vi "CheckDayPassing.vi"(8 "error in":errorcluster, 10 "Data2save.time":dbl[](array[numeric]), 11 "TableName":string) -> (0 "error out":errorcluster, 1 "split-index":i32, 2 "Split array":bool, 3 "FolderPace":T1, 4 "TimeValid":bool, 5 "PeriodName2":string, 7 "PeriodName1":string)   [LabVIEW 2020, in "Sgraph_lib_V1.lvlib" / "DBAL-BIN.lvclass"]
doc: "This VI will check if the time of the dataset is passing one period.\nIf that is the case, then the dataset has to be split in two subsections and processed separately.\n\nAlthough the name of this routine is called 'DayPassing' this was later changed to 'one week' or 'one year' for other file types. Therefore this VI actually checks if the period is passed for which a new file is needed."
uses:
  DBAL-BIN.lvclass
  BinFolderPace.ctl
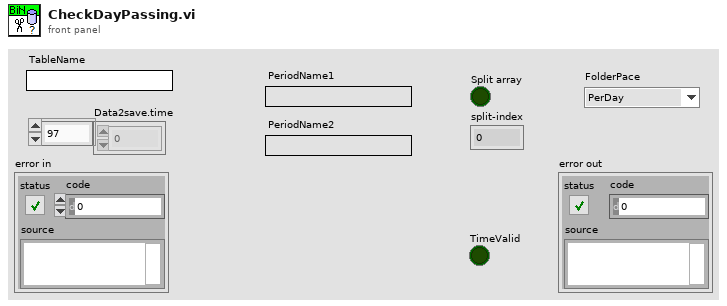
[diagram p1: front panel]
types:
  T1 = typedef "Sgraph_lib_V1.lvlib/DBAL-BIN.lvclass/BinFolderPace.ctl" = enum16{"PerDay", "PerWeek", "PerYear"}
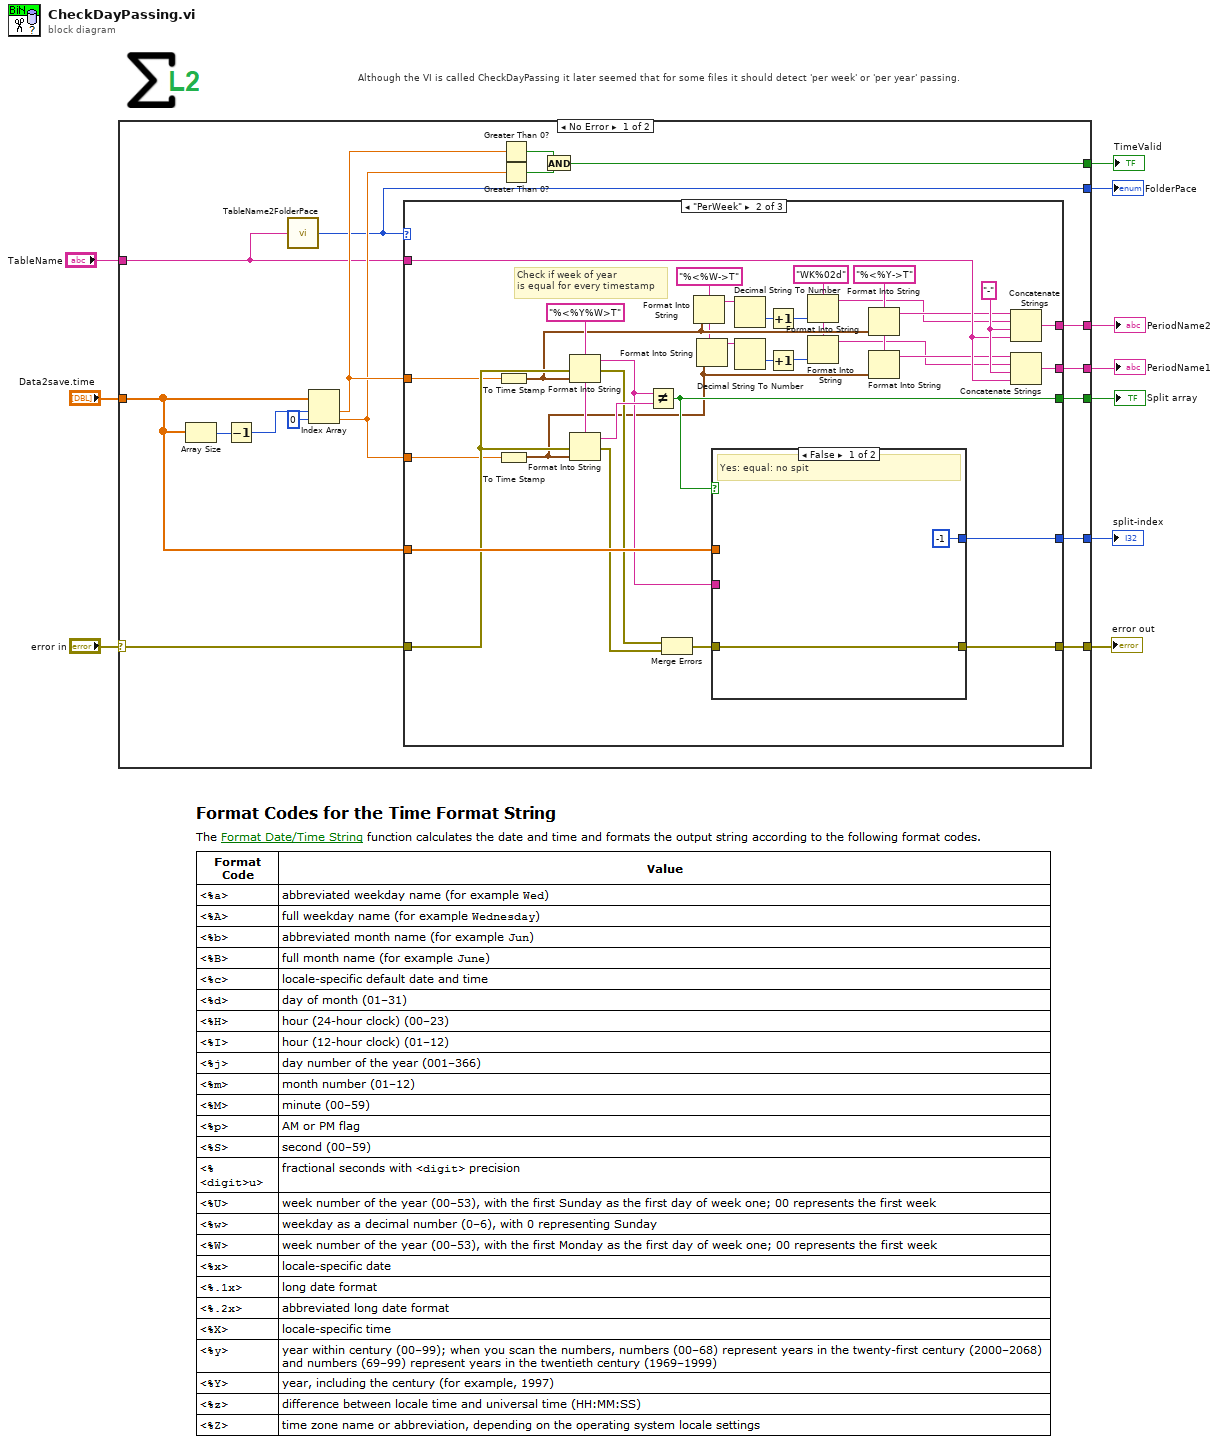
[diagram p0: block diagram]
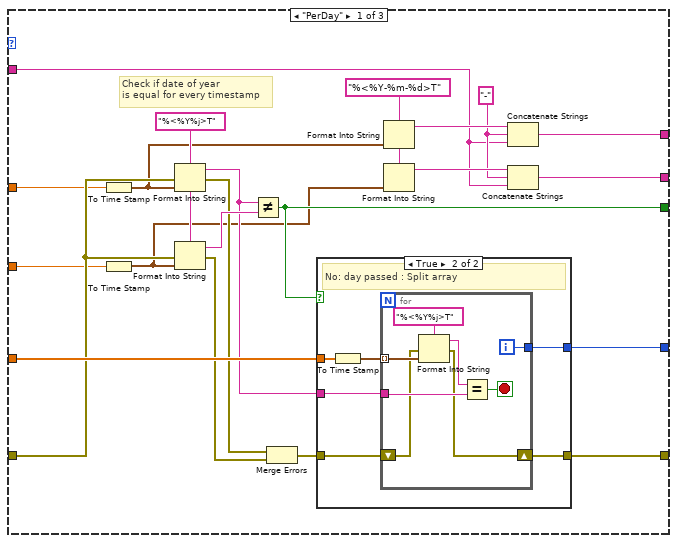
[diagram p2: hidden frame]
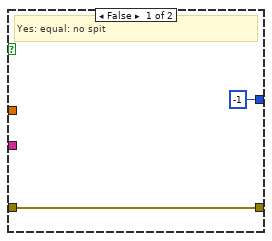
[diagram p3: hidden frame]
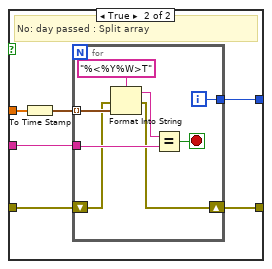
[diagram p4: hidden frame]
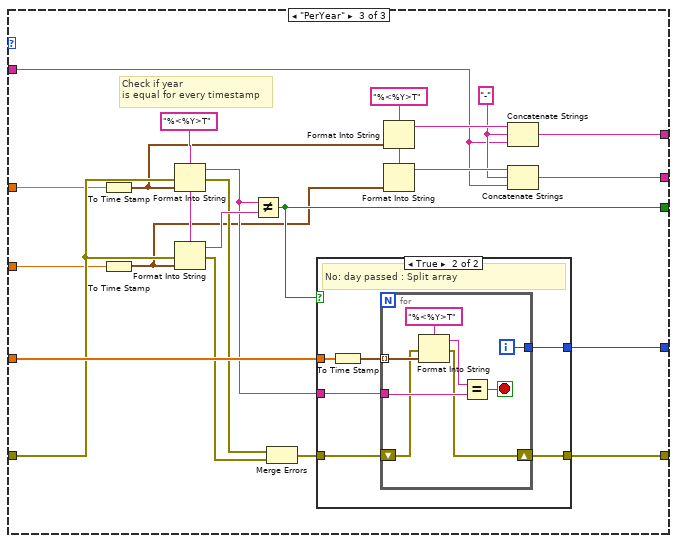
[diagram p5: hidden frame]
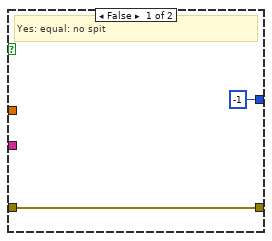
[diagram p6: hidden frame]
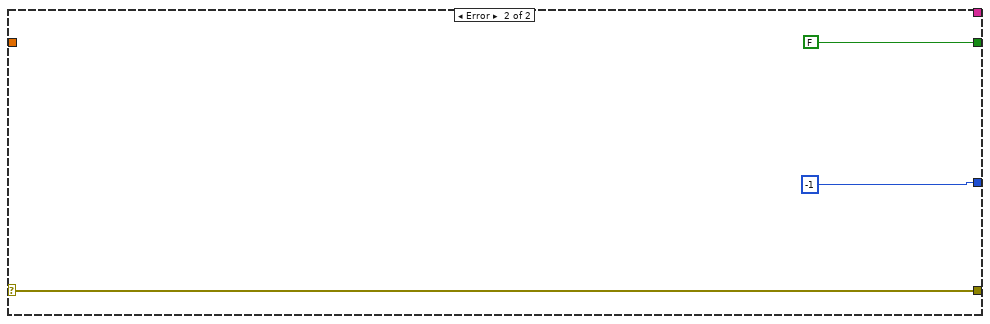
[diagram p7: hidden frame]
diagram:
  # "Although the VI is called CheckDayPassing it later seemed that for some files it should detect 'per week' or 'per year' passing."
  n1 = case shown="No Error" "error in" {
    selector: "error in" -> [w21 w154]
    tunnel: "Data2save.time" -> [w24 _]
    tunnel: [w23 -1] -> w9
    tunnel: [w22 w154] -> w8
    tunnel: [w20 FALSE] -> w6
    tunnel: [w19 _] -> w5
    tunnel: [w18 _] -> w4
    tunnel: "TableName" -> [w12 _]
    tunnel: [w13 _] -> w2
    tunnel: [w11 _] -> w1
    frame No Error {
      n2 = Array Size(array=w24) -> (size(s)=w27:i32)
      n3 = Decrement(x=w27) -> (x-1=w26:i32)
      n4 = call "TableName2FolderPace.vi"("TableName"=w12) -> ("FolderPace"=w11:T1)  [unwired: 6 in]
      n5 = Index Array(array=w24, index #1=w26, index #2=0 ("index")) -> (element #1=w17:dbl, element #2=w16:dbl)
      n6 = case shown="\"PerWeek\"" w11 {
        tunnel: w24 -> [w48 w96 w134]
        tunnel: [w46 w94 w132] -> w23
        tunnel: [w41 w89 w127] -> w22
        tunnel: w21 -> [w40 w88 w126]
        tunnel: [w39 w87 w125] -> w20
        tunnel: [w32 w84 w118] -> w19
        tunnel: [w31 w83 w117] -> w18
        tunnel: w17 -> [w30 w82 w116]
        tunnel: w16 -> [w29 w81 w115]
        tunnel: w12 -> [w28 w80 w114]
        frame "PerDay" {
          w33 = "-" ("initial string")
          w36 = "%<%Y-%m-%d>T" ("format string")
          w49 = "%<%Y%j>T" ("format string")
          # "Check if date of year\nis equal for every timestamp"
          n7 = To Time Stamp(1:w30) -> (0:w37:timestamp)
          n8 = To Time Stamp(1:w29) -> (0:w38:timestamp)
          n9 = Format Into String(format string=w49, error in=w40, w37) -> (resulting string=w45:string, error out=w44:errorcluster)  [unwired: 1 in]
          n10 = Format Into String(format string=w49, error in=w40, w38) -> (resulting string=w47:string, error out=w43:errorcluster)  [unwired: 1 in]
          n11 = Not Equal?(x=w45, y=w47) -> (x != y?=w39:bool)
          n12 = Merge Errors(w44, w43) -> (w42:errorcluster)
          n13 = case shown="True" w39 {
            tunnel: w48 -> [_ w57]
            tunnel: w45 -> [_ w55]
            tunnel: [-1 w54] -> w46
            tunnel: w42 -> [w50 w53]
            tunnel: [w50 w52] -> w41
            frame False {
              # "Yes: equal: no spit"
            }
            frame True {
              # "No: day passed : Split array"
              n14 = To Time Stamp(1:w57) -> (0:w56:timestamp[])
              n15 = for {
                tunnel: w56 -> [w64] mode=indexing
                tunnel: w55 -> [w62]
                tunnel: [w60] -> w54
                shift-right: [w58] -> w52
                shift-left: w53 -> [w59]
                i -> [w60]
                stop <- w61 stop-if-true
                n16 = Format Into String(format string="%<%Y%j>T", error in=w59, w64) -> (resulting string=w63:string, error out=w58:errorcluster)  [unwired: 1 in]
                n17 = Equal?(x=w63, y=w62) -> (x = y?=w61:bool)
              }
            }
          }
          n18 = Format Into String(format string=w36, w37) -> (resulting string=w35:string)  [unwired: 2 in, 1 out]
          n19 = Format Into String(format string=w36, w38) -> (resulting string=w34:string)  [unwired: 2 in, 1 out]
          n20 = Concatenate Strings(w35, w33, w28) -> (w32:string)
          n21 = Concatenate Strings(w34, w33, w28) -> (w31:string)
        }
        frame "PerWeek" {
          w70 = "WK%02d" ("format string")
          w77 = "%<%W->T" ("format string")
          w85 = "-" ("initial string")
          w86 = "%<%Y->T" ("format string")
          w97 = "%<%Y%W>T" ("format string")
          # "Check if week of year\nis equal for every timestamp"
          n22 = To Time Stamp(1:w82) -> (0:w79:timestamp)
          n23 = To Time Stamp(1:w81) -> (0:w78:timestamp)
          n24 = Format Into String(format string=w97, error in=w88, w79) -> (resulting string=w93:string, error out=w92:errorcluster)  [unwired: 1 in]
          n25 = Format Into String(format string=w97, error in=w88, w78) -> (resulting string=w95:string, error out=w91:errorcluster)  [unwired: 1 in]
          n26 = Not Equal?(x=w93, y=w95) -> (x != y?=w87:bool)
          n27 = Merge Errors(w92, w91) -> (w90:errorcluster)
          n28 = Format Into String(format string=w77, w79) -> (resulting string=w76:string)  [unwired: 2 in, 1 out]
          n29 = Format Into String(format string=w77, w78) -> (resulting string=w75:string)  [unwired: 2 in, 1 out]
          n30 = case shown="False" w87 {
            tunnel: w96 -> [_ w105]
            tunnel: w93 -> [_ w103]
            tunnel: [-1 w102] -> w94
            tunnel: w90 -> [w98 w101]
            tunnel: [w98 w100] -> w89
            frame False {
              # "Yes: equal: no spit"
            }
            frame True {
              # "No: day passed : Split array"
              n31 = To Time Stamp(1:w105) -> (0:w104:timestamp[])
              n32 = for {
                tunnel: w104 -> [w112] mode=indexing
                tunnel: w103 -> [w110]
                tunnel: [w108] -> w102
                shift-right: [w106] -> w100
                shift-left: w101 -> [w107]
                i -> [w108]
                stop <- w109 stop-if-true
                n33 = Format Into String(format string="%<%Y%W>T", error in=w107, w112) -> (resulting string=w111:string, error out=w106:errorcluster)  [unwired: 1 in]
                n34 = Equal?(x=w111, y=w110) -> (x = y?=w109:bool)
              }
            }
          }
          n35 = Decimal String To Number(string=w76) -> (number=w74:i32)  [unwired: 2 in, 1 out]
          n36 = Decimal String To Number(string=w75) -> (number=w73:i32)  [unwired: 2 in, 1 out]
          n37 = Increment(x=w74) -> (x+1=w72:i32)
          n38 = Increment(x=w73) -> (x+1=w71:i32)
          n39 = Format Into String(format string=w70, w72) -> (resulting string=w67:string)  [unwired: 2 in, 1 out]
          n40 = Format Into String(format string=w70, w71) -> (resulting string=w66:string)  [unwired: 2 in, 1 out]
          n41 = Format Into String(format string=w86, w79) -> (resulting string=w68:string)  [unwired: 2 in, 1 out]
          n42 = Format Into String(format string=w86, w78) -> (resulting string=w69:string)  [unwired: 2 in, 1 out]
          n43 = Concatenate Strings(w68, w67, w85, w80) -> (w84:string)
          n44 = Concatenate Strings(w69, w66, w85, w80) -> (w83:string)
        }
        frame "PerYear" {
          w119 = "-" ("initial string")
          w122 = "%<%Y>T" ("format string")
          w135 = "%<%Y>T" ("format string")
          # "Check if year\nis equal for every timestamp"
          n45 = To Time Stamp(1:w116) -> (0:w123:timestamp)
          n46 = To Time Stamp(1:w115) -> (0:w124:timestamp)
          n47 = Format Into String(format string=w135, error in=w126, w123) -> (resulting string=w131:string, error out=w130:errorcluster)  [unwired: 1 in]
          n48 = Format Into String(format string=w135, error in=w126, w124) -> (resulting string=w133:string, error out=w129:errorcluster)  [unwired: 1 in]
          n49 = Not Equal?(x=w131, y=w133) -> (x != y?=w125:bool)
          n50 = Merge Errors(w130, w129) -> (w128:errorcluster)
          n51 = case shown="True" w125 {
            tunnel: w134 -> [_ w143]
            tunnel: w131 -> [_ w141]
            tunnel: [-1 w140] -> w132
            tunnel: w128 -> [w136 w139]
            tunnel: [w136 w138] -> w127
            frame False {
              # "Yes: equal: no spit"
            }
            frame True {
              # "No: day passed : Split array"
              n52 = To Time Stamp(1:w143) -> (0:w142:timestamp[])
              n53 = for {
                tunnel: w142 -> [w150] mode=indexing
                tunnel: w141 -> [w148]
                tunnel: [w146] -> w140
                shift-right: [w144] -> w138
                shift-left: w139 -> [w145]
                i -> [w146]
                stop <- w147 stop-if-true
                n54 = Format Into String(format string="%<%Y>T", error in=w145, w150) -> (resulting string=w149:string, error out=w144:errorcluster)  [unwired: 1 in]
                n55 = Equal?(x=w149, y=w148) -> (x = y?=w147:bool)
              }
            }
          }
          n56 = Format Into String(format string=w122, w123) -> (resulting string=w121:string)  [unwired: 2 in, 1 out]
          n57 = Format Into String(format string=w122, w124) -> (resulting string=w120:string)  [unwired: 2 in, 1 out]
          n58 = Concatenate Strings(w121, w119, w114) -> (w118:string)
          n59 = Concatenate Strings(w120, w119, w114) -> (w117:string)
        }
      }
      n60 = Greater Than 0?(x=w17) -> (x > 0?=w15:bool)
      n61 = Greater Than 0?(x=w16) -> (x > 0?=w14:bool)
      n62 = And(x=w15, y=w14) -> (x .and. y?=w13:bool)
    }
    frame Error {
    }
  }
  "split-index" <- w9
  "error out" <- w8
  "Split array" <- w6
  "PeriodName1" <- w4
  "PeriodName2" <- w5
  "TimeValid" <- w2
  "FolderPace" <- w1
